vi "LVImageDataToPNGByteArray Wrapper Template.vi"(0 "compression":i32=1, 1 "width":u32, 2 "height":u32, 3 "depth":i32=24, 4 "imageBuf":u8[](array[numeric]), 5 "colorTable":i32[](array[numeric]), 6 "colorTableSize":i32, 7 "error in":errorcluster) -> (20 "png data":u8[](array[numeric]), 27 "error out":errorcluster)   [LabVIEW 2020]
doc: "Encodes raw LabVIEW image data as a PNG file in memory, through LVImageDataToPNGByteArray, the function LabVIEW itself exports (library LabVIEW, C calling convention, called in any thread) and NI's LV Image to PNG Data.vi calls. Unlike that VI it takes the zlib level in every LabVIEW version: LabVIEW 2020's copy of it has no compression input and always writes an uncompressed PNG. compression is the zlib level: 0 none, 1 fastest, 9 smallest, -1 zlib's default; above 9 the function returns an empty png and no error. When error in carries an error the function is not called. Generated by tools\\Build Win32 Wrappers.vi - do not edit by hand, rebuild it."
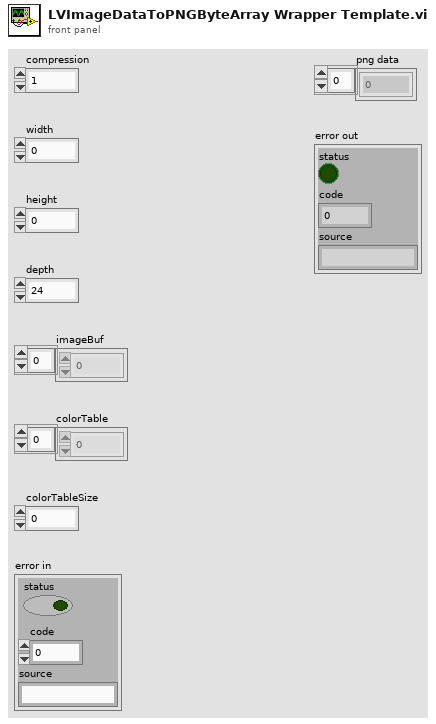
[diagram p1: front panel]
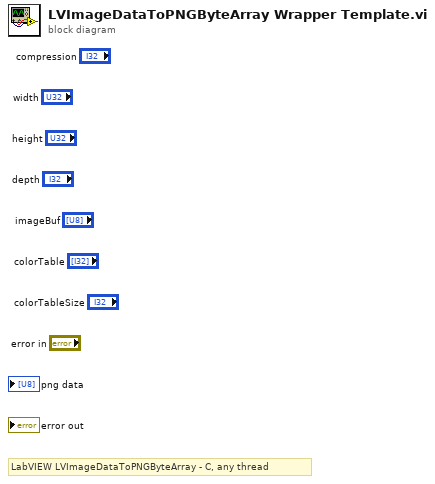
[diagram p0: block diagram]
diagram:
  # "LabVIEW LVImageDataToPNGByteArray - C, any thread"
